vi "ZM-HW-init.vi"(8 "error in (no error)":errorcluster, 11 "ZM-HW-hardware in":refnum<class "ZM-HW-hardware.lvclass">) -> (0 "error out":errorcluster, 3 "ZM-HW-hardware out":refnum<class "ZM-HW-hardware.lvclass">)   [LabVIEW 2020, in "ZM-HW-hardware.lvlib" / "ZM-HW-hardware.lvclass"]
doc: "Initialises the hardware object (dynamic dispatch): writes initialized = TRUE through the private accessor Write initialized. This is the real default of the parent; a child may override it and call the parent."
uses:
  ZM-HW-hardware.lvclass
  ZM-HW-hardware.lvclass/ZM-HW-hardware.ctl
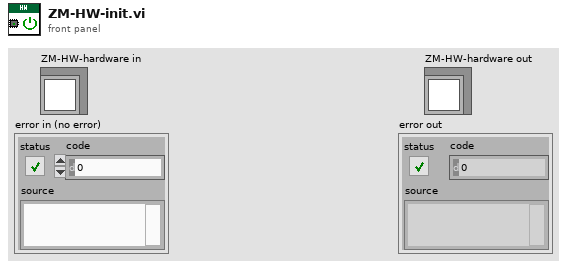
[diagram p1: front panel]
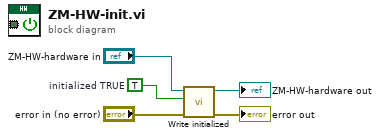
[diagram p0: block diagram]
diagram:
  w3 = TRUE  # initialized TRUE
  n1 = call "Write initialized.vi"("error in (no error)"="error in (no error)", "initialized"=w3, "ZM-HW-hardware in"="ZM-HW-hardware in") -> ("error out"=→"error out":errorcluster, "ZM-HW-hardware out"=→"ZM-HW-hardware out":refnum<class "ZM-HW-hardware.lvclass">)  [unwired: 7 in]
